vi "set Velocity.vi"(8 "error in (no error)":errorcluster, 10 "Velocity (degree/sec)":dbl, 11 "3D Controller in":refnum<class "3D Controller.lvclass">) -> (0 "error out":errorcluster, 3 "3D Controller out":refnum<class "3D Controller.lvclass">)   [LabVIEW 2023, in "FCC 3D Controller for BS.lvlib" / "3D Controller.lvclass"]
uses:
  3D Controller.lvclass
  3D Controller.lvclass/3D Controller.ctl
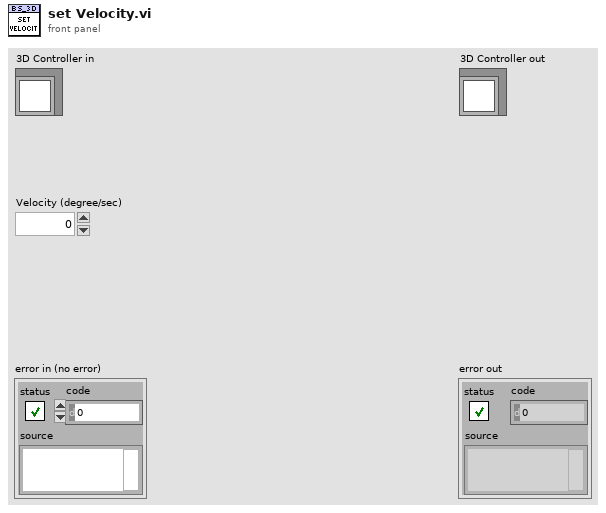
[diagram p1: front panel]
types:
  T1 = typedef "FCC 3D Controller for BS.lvlib/TYPE Protocol Char of Command.ctl" = cluster{"Header":string, "Axis No.":i32, "End":string}
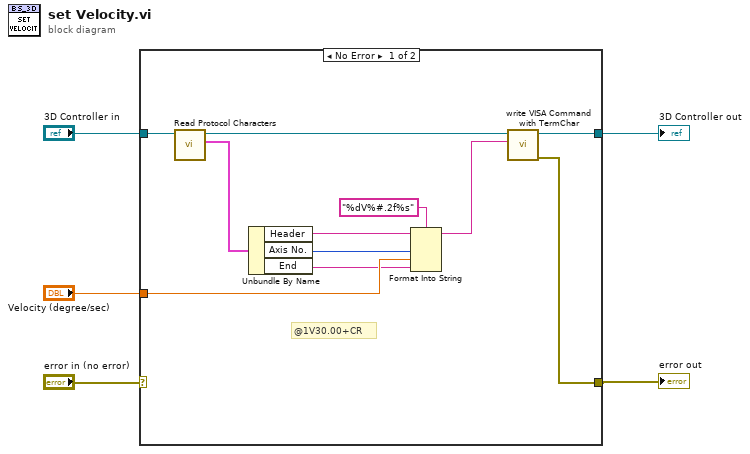
[diagram p0: block diagram]
diagram:
  n1 = case shown="No Error" "error in (no error)" {
    selector: "error in (no error)" -> [_ w18]
    tunnel: "3D Controller in" -> [w6 w17]
    tunnel: [w7 w18] -> w1
    tunnel: [w9 w17] -> w4
    tunnel: "Velocity (degree/sec)" -> [w12 _]
    frame No Error {
      # "@1V30.00+CR"
      n2 = call "Read Protocol Characters.vi"("3D Controller in"=w6) -> ("Protocol Characters"=w15:T1, "3D Controller out"=w10:refnum<class "3D Controller.lvclass">)  [unwired: 8 in, 1 out]
      n3 = Unbundle By Name(w15) -> ("Header"=w14:string, "Axis No."=w13:i32, "End"=w11:string)
      n4 = Format Into String(format string="%dV%#.2f%s", initial string=w14, w13, w12, w11) -> (resulting string=w8:string)  [unwired: 1 in, 1 out]
      n5 = call "write VISA Command with TermChar.vi"("Command String"=w8, "3D Controller in"=w10) -> ("error out"=w7:errorcluster, "3D Controller out"=w9:refnum<class "3D Controller.lvclass">)  [unwired: 8 in]
    }
    frame Error {
    }
  }
  "error out" <- w1
  "3D Controller out" <- w4
